vi "RemoteVI Read Panel Info.vi"(0 "VI":refnum<vi>, 1 "hWnd":u64, 2 "refresh?":bool, 3 "origin":cluster{"x":i32, "y":i32}, 5 "tips in":string="tips []", 6 "splitters in":string="splitters []", 7 "bars in":T1(array[cluster])) -> (4 "tips out":string, 8 "splitters out":string, 9 "bars out":T1(array[cluster]))   [LabVIEW 2020, in "RemoteVI.lvlib"]
doc: "The tip strips and splitter bars of the published panel (tips and splitters messages, docs\\protocol.md 3.3) when refresh? is TRUE. A panel of this LabVIEW: RemoteVI Read Tips.vi and RemoteVI Read Splitters.vi. A panel of another LabVIEW reached over VI Server (RemoteVI Remote Target.vi has an entry for hWnd): both run INSIDE that process through RemoteVI Remote Hooks.vi (RemoteVI Call Hooks.vi) - one round trip of a few VI Server calls instead of one per control, and the pane coordinate conversions stay in the process that owns the panes. Otherwise, or on an error, the inputs pass through."
uses:
  RemoteVI.lvlib
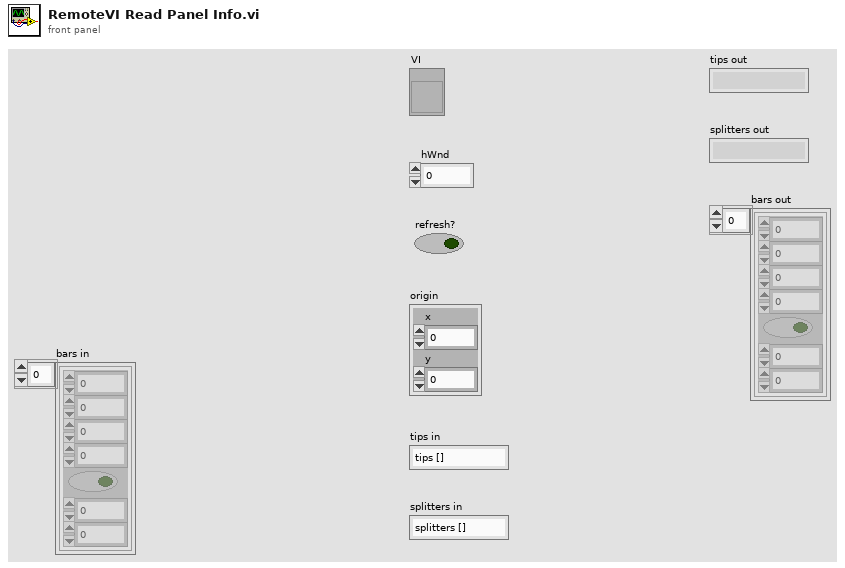
[diagram p1: front panel]
types:
  T1 = cluster{"x":i32, "y":i32, "w":i32, "h":i32, "vertical":bool, "min":i32, "max":i32}[]
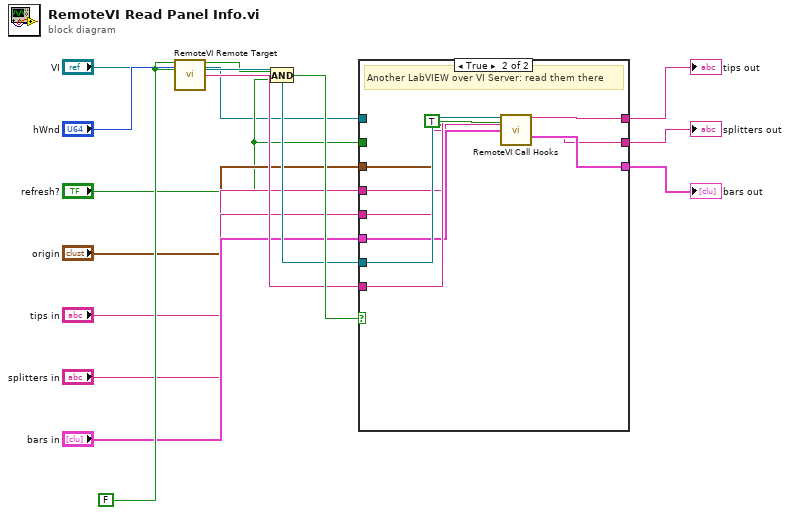
[diagram p0: block diagram]
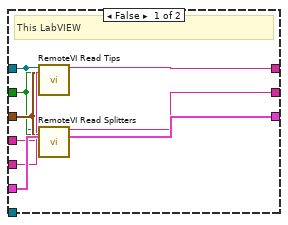
[diagram p2: hidden frame]
diagram:
  w8 = FALSE
  n1 = call "RemoteVI Remote Target.vi"("put?"=w8, "hWnd"="hWnd", "remove?"=w8) -> ("found?"=w9:bool, "hooks out"=w10:refnum<vi>, "VI name out"=w11:string)  [unwired: 10 in]
  n2 = And(x=w9, y="refresh?") -> (x .and. y?=w12:bool)
  n3 = case shown="True" w12 {
    tunnel: "VI" -> [w16 _]
    tunnel: "refresh?" -> [w17 _]
    tunnel: "origin" -> [w18 w25]
    tunnel: "tips in" -> [w19 w26]
    tunnel: "splitters in" -> [w20 w27]
    tunnel: "bars in" -> [w21 w28]
    tunnel: w10 -> [_ w29]
    tunnel: w11 -> [_ w30]
    tunnel: [w22 w32] -> w13
    tunnel: [w23 w33] -> w14
    tunnel: [w24 w34] -> w15
    frame False {
      # "This LabVIEW"
      n4 = call "RemoteVI Read Tips.vi"("VI"=w16, "refresh?"=w17, "origin"=w18, "message in"=w19) -> ("message out"=w22:string)  [unwired: 11 in]
      n5 = call "RemoteVI Read Splitters.vi"("VI"=w16, "refresh?"=w17, "origin"=w18, "message in"=w20, "bars in"=w21) -> ("message out"=w23:string, "bars out"=w24:T1)  [unwired: 9 in]
    }
    frame True {
      # "Another LabVIEW over VI Server: read them there"
      n6 = call "RemoteVI Call Hooks.vi"("hooks"=w29, "panel?"=TRUE, "VI name"=w30, "origin"=w25, "tips in"=w26, "splitters in"=w27, "bars in"=w28) -> ("tips out"=w32:string, "splitters out"=w33:string, "bars out"=w34:T1)  [unwired: 5 in, 1 out]
    }
  }
  "tips out" <- w13
  "splitters out" <- w14
  "bars out" <- w15
